vi "MQTT Data - Decode Byte.vi"(5 "remaining data in":u8[](array[numeric])) -> (1 "U8":u8, 2 "remaining data out":u8[](array[numeric]))   [LabVIEW 2019, in "KoRE-MQTT.lvlib"]
doc: "Copyright (c) 2025 KoRElibs.com\nSPDX-License-Identifier: EUPL-1.2\n\nThis VI is licensed under the European Union Public License (EUPL) Version 1.2. You may use this VI unmodified in proprietary works. If you distribute a modified version of this file, the modified file must be released under the EUPL-1.2. Full license: https://joinup.ec.europa.eu/asset/eupl/eupl/1.2/"
uses:
  KoRE-MQTT.lvlib
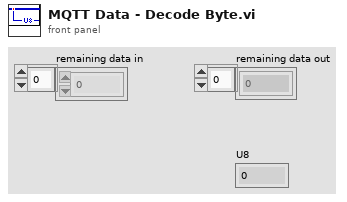
[diagram p1: front panel]
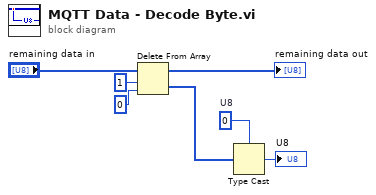
[diagram p0: block diagram]
diagram:
  w6 = u8 0  # U8
  n1 = Delete From Array(array="remaining data in", length=1, index=0) -> (deleted portion=w5:u8[], array with subset deleted=→"remaining data out":u8[])
  n2 = Type Cast(type=w6, x=w5) -> (*(type *) &x=→"U8":u8)
